vi "Create Cache.vi"() -> (3 "ConfigManager.Cache":refnum<class "ConfigManager.Cache.lvclass">)   [LabVIEW 2013, in "CfgManager.lvlib" / "ConfigManager.Cache.lvclass"]
uses:
  ConfigManager.Cache.lvclass
  ConfigManager.Cache.lvclass/ConfigManager.Cache.ctl
  Manager/ConfigManager.lvclass/ConfigManager.ctl
  Manager/ConfigManager.lvclass
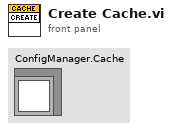
[diagram p1: front panel]
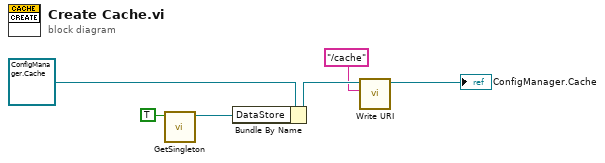
[diagram p0: block diagram]
diagram:
  n1 = call "GetSingleton.vi"("Creator (F)"=TRUE) -> ("DataStore"=w5:refnum<data-value>)  [unwired: 9 in, 1 out]
  n2 = Bundle By Name(cluster=refnum<class "ConfigManager.Cache.lvclass"> refnum ("ConfigManagerCollection.lvclass"), "DataStore"=w5) -> (w3:refnum<class "ConfigManager.Cache.lvclass">)
  n3 = call "Write URI.vi"("URI"="/cache", "ConfigManager in"=w3) -> ("ConfigManager out"=→"ConfigManager.Cache":refnum<class "ConfigManager.Cache.lvclass">)  [unwired: 9 in]
